vi "Write.vi"(8 "error in (no error)":errorcluster, 9 "timeout (ms)":i32=1000, 10 "pcap CAN DATA in":u8[](array[numeric]), 11 "CAN RW CANsub in":refnum<class "CAN RW CANsub.lvclass">) -> (0 "error out":errorcluster, 3 "CAN RW CANsub out":refnum<class "CAN RW CANsub.lvclass">, 4 "number written":i32=-1)   [LabVIEW 2021, in "CAN RW CANsub.lvclass"]
doc: "Sends pcap CAN packets as CAN frames with one TCP Write. Remote frames and error frames are not sent and are counted as filtered frames. After the send, it reads the transmit acknowledgements from the socket with timeout 0. Error 5302 if not all bytes were converted. Phase 1: timeout (ms) and One Shot TX are not used, and ACK Errors is 0. Loop-safe: no allocation in this class, bounded time (TCP Write timeout 1 s)."
uses:
  CAN RW CANsub.lvclass
  C:/Program Files/National Instruments/LabVIEW 2025/vi.lib/CIF Foundation/CIF CAN RW Core/CAN_RW_CORE.lvclass
  CAN RW CANsub.lvclass/CAN RW CANsub.ctl
  <vilib>/CIF Foundation/CIF CAN RW Core/CAN_RW_CORE.lvclass/CAN_RW_CORE.ctl
  CANsub/c_client/api/CANsub_Channel/CANsub_Channel.lvclass
  CANsub/c_client/CANsub_C.lvlib
  <vilib>/CIF Foundation/CIF CAN RW Core/CAN_RW_CORE.lvclass
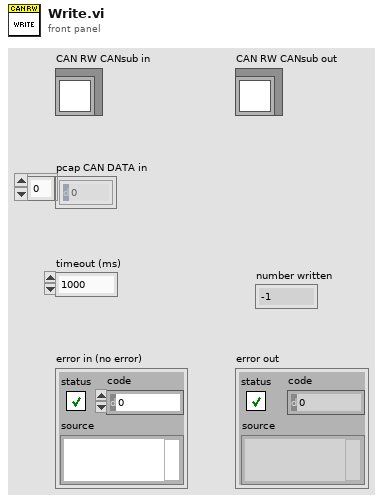
[diagram p1: front panel]
types:
  T1 = typedef "CANsub_API.lvlib/CANsub_Frames.ctl" = cluster{"count":i32, "t_dev":dbl[], "id":u32[], "flags":u16[], "dlc":u8[], "data len":u8[], "data":u8[]}
  T2 = typedef "CANsub_API.lvlib/CANsub_Pcap_Options.ctl" = cluster{"allow list":u32[], "deny list":u32[], "TAI minus UTC (s)":i32, "keep TX acks":bool, "little endian":bool}
  T3 = typedef "CANsub_C.lvlib/C_CIF_Encode_Result.ctl" = cluster{"length":i32, "n packets":i32, "n rejected":i32, "consumed":i32}
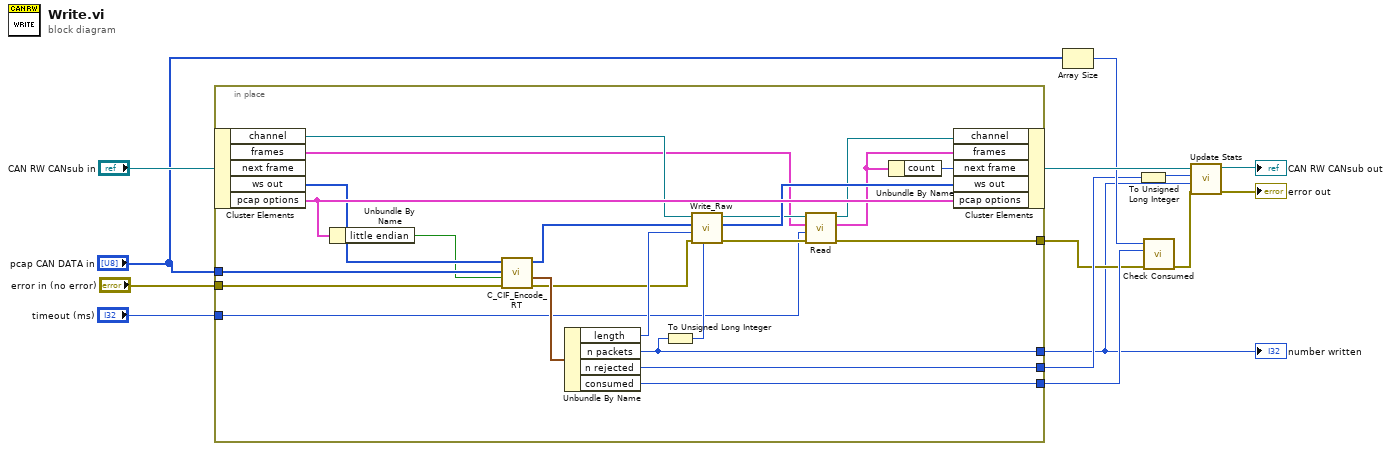
[diagram p0: block diagram]
diagram:
  n1 = in-place {
    in-place-border: "pcap CAN DATA in" -> [w35]
    in-place-border: "error in (no error)" -> [w33]
    in-place-border: "timeout (ms)" -> [w22]
    in-place-border: [w18] -> w7
    in-place-border: [w17] -> w5
    in-place-border: [w16] -> w4
    in-place-border: [w15] -> w1
    n2 = in-place-cluster #1("CAN RW CANsub in") -> ("channel"=w31:refnum<class "CANsub_Channel.lvclass">, "frames"=w24:T1, "ws out"=w36:u8[], "pcap options"=w37:T2)  [unwired: 1 out]
    n3 = Unbundle By Name(w37) -> ("little endian"=w34:bool)
    n4 = call "C_CIF_Encode_RT.vi"("error in (no error)"=w33, "little endian"=w34, "pcap"=w35, "tx in"=w36) -> ("error out"=w27:errorcluster, "result"=w32:T3, "tx out"=w30:u8[])  [unwired: 5 in]
    n5 = Unbundle By Name(w32) -> ("length"=w29:i32, "n packets"=w15:i32, "n rejected"=w17:i32, "consumed"=w18:i32)
    n6 = To Unsigned Long Integer(number=w15) -> (unsigned 32bit integer=w28:u32)
    n7 = call-dynamic "Write_Raw.vi"("n frames"=w28, "error in (no error)"=w27, "length"=w29, "bytes in"=w30, "channel in"=w31) -> ("error out"=w23:errorcluster, "bytes out"=w26:u8[], "channel out"=w25:refnum<class "CANsub_Channel.lvclass">)  [unwired: 4 in]
    n8 = call-dynamic "Read.vi"("error in (no error)"=w23, "timeout ms"=w22, "frames in"=w24, "channel in"=w25) -> ("error out"=w16:errorcluster, "frames out"=w20:T1, "channel out"=w21:refnum<class "CANsub_Channel.lvclass">)  [unwired: 5 in]
    n9 = Unbundle By Name(w20) -> ("count"=w19:i32)
    n10 = in-place-cluster #1("channel"=w21, "frames"=w20, "next frame"=w19, "ws out"=w26, "pcap options"=w37) -> (w10:refnum<class "CAN RW CANsub.lvclass">)
  }
  "number written" <- w1
  n11 = Array Size(array="pcap CAN DATA in") -> (size(s)=w8:i32)
  n12 = To Unsigned Long Integer(number=w5) -> (unsigned 32bit integer=w6:u32)
  n13 = call "Check Consumed.vi"("error in (no error)"=w4, "consumed"=w7, "size"=w8) -> ("error out"=w3:errorcluster)  [unwired: 8 in]
  n14 = call <vilib>:"Update Stats.vi"("error in (no error)"=w3, "Number Read"=w1, "Number Filtered"=w6, "CAN_RW_CORE in"=w10) -> ("error out"=→"error out":errorcluster, "CAN_RW_CORE out"=→"CAN RW CANsub out":refnum<class "CAN RW CANsub.lvclass">)  [unwired: 6 in]
